vi "Set PWM Dutty Cycle.vi"   [LabVIEW 2020, in "wiringPi.lvlib"]
doc: "<b>_______________________________________________________________</b>\n** Author: Juan José Villacorta\n** LabVIEW wrapper for C library <b> wiringPi </b>,\n** https://github.com/WiringPi/WiringPi\n<b>_______________________________________________________________</b>\n\nConfigure a GPIO Pin as PWM output"
uses:
  wiringPi.lvlib
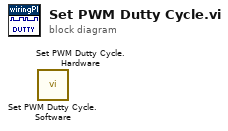
[diagram p0: block diagram]
diagram:
  n1 = call "Set PWM Dutty Cycle.Software.vi"() -> ()  [unwired: 10 in, 2 out]
  n2 = call "Set PWM Dutty Cycle.Hardware.vi"() -> ()  [unwired: 10 in, 2 out]
